vi "Build_Asylum_GetRange.vi"(8 "error in (no error)":errorcluster, 11 "parameterName":string) -> (0 "error out":errorcluster, 3 "Command":string)   [LabVIEW 2019]
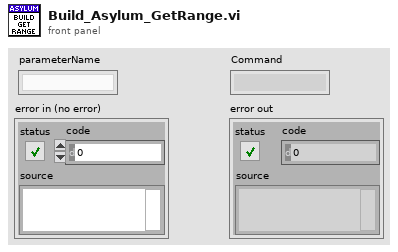
[diagram p1: front panel]
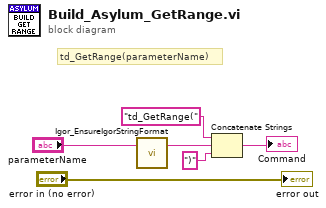
[diagram p0: block diagram]
diagram:
  # "td_GetRange(parameterName)"
  n1 = call <userlib>:"Igor_EnsureIgorStringFormat.vi"("Value"="parameterName") -> ("Value"=w4:string)  [unwired: 2 in]
  n2 = Concatenate Strings("td_GetRange(" ("string"), w4, ")" ("string")) -> (→"Command":string)
  "error out" <- "error in (no error)"
